vi "Resubscribe to Cloneable.vi"(8 "error in":errorcluster, 11 "Module ID":i32=-1) -> (0 "error out":errorcluster)   [LabVIEW 2026, in "Core.lvlib"]
doc: "_____\nCreated using DQMH Framework: Event Scripter 7.1.2.1547."
uses:
  Core.lvlib
  Resubscribe to Cloneable Argument--cluster.ctl
  replay/Replay/src/Libraries/Replay/Broadcast Events--cluster.ctl
  replay/Replay/src/Libraries/Replay/Did Init Argument--cluster.ctl
  replay/Replay/src/Libraries/Replay/Status Updated Argument--cluster.ctl
  replay/Replay/src/Libraries/Replay/Error Reported Argument--cluster.ctl
  replay/Replay/src/Libraries/Replay/Stop Argument--cluster.ctl
  replay/Replay/src/Libraries/Replay/Get Module Execution Status Argument--cluster.ctl
  replay/Replay/src/Libraries/Replay/Replay Finished Processing User Events Argument--cluster.ctl
  replay/Replay/src/Libraries/Replay/Load UserEvents (Reply Payload)--cluster.ctl
  replay/Replay/src/Libraries/User Events Metadata.ctl
  replay/Replay/src/Libraries/Replay/Replay.lvlib
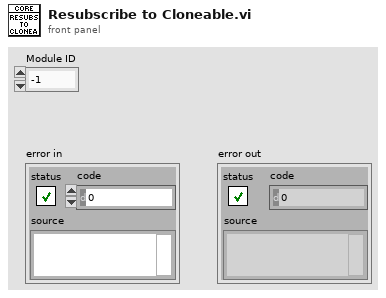
[diagram p1: front panel]
types:
  T1 = typedef "Replay.lvlib/Broadcast Events--cluster.ctl" = cluster{"Module Did Init":refnum<user-event>, "Status Updated":refnum<user-event>, "Error Reported":refnum<user-event>, "Module Did Stop":refnum<user-event>, "Update Module Execution Status":refnum<user-event>, "Replay Finished Processing User Events":refnum<user-event>, "User Events Metadata":refnum<user-event>}
  T2 = typedef "Core.lvlib/Resubscribe to Cloneable Argument--cluster.ctl" = cluster{"Module ID":i32, "Replay Broadcast Events":T1}
  T3 = typedef "Core.lvlib/Request Events--cluster.ctl" = cluster{"Stop Module":refnum<user-event>, "Show Panel":refnum<user-event>, "Hide Panel":refnum<user-event>, "Show Diagram":refnum<user-event>, "Get Module Execution Status":refnum<user-event>, "Resubscribe to Cloneable":refnum<user-event>, "LaunchReplayModule":refnum<user-event>, "Local Instance":T4, "Record Run ID":refnum<user-event>}
  T4 = typedef "Core.lvlib/Local Instance Request Events--cluster.ctl" = cluster{"Set Record Run ID":refnum<user-event>}
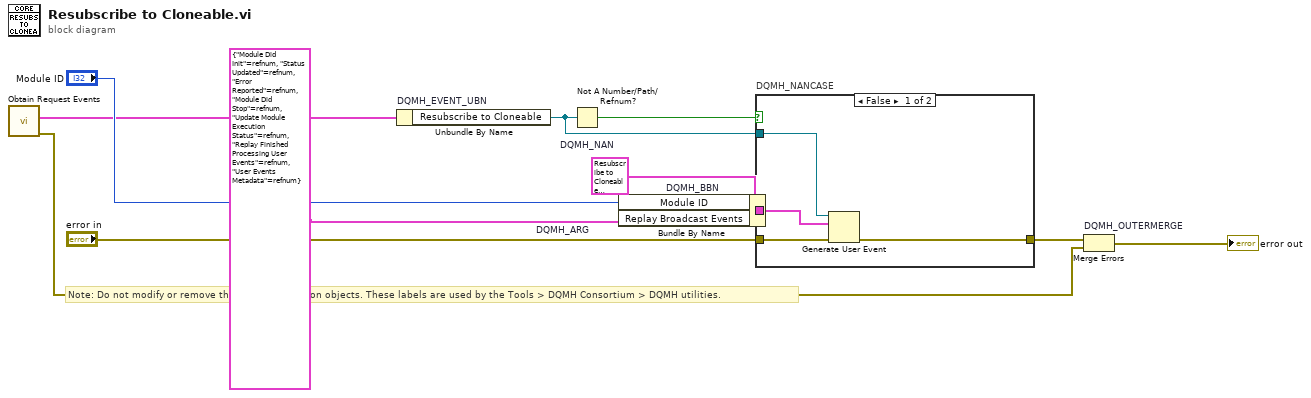
[diagram p0: block diagram]
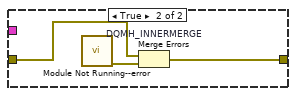
[diagram p2: hidden frame]
diagram:
  w5 = T2 {"Module ID"=-1, "Replay Broadcast Events"={"Module Did Init"=refnum, "Status Updated"=refnum, "Error Reported"=refnum, "Module Did Stop"=refnum, "Update Module Execution Status"=refnum, "Replay Finished Processing User Events"=refnum, "User Events Metadata"=refnum}}  # DQMH_ARG
  # "Note: Do not modify or remove the \"DQMH\" labels on objects. These labels are used by the Tools > DQMH Consortium > DQMH utilities."
  n1 = call "Obtain Request Events.vi"() -> ("error out"=w3:errorcluster, "Core Request Events"=w2:T3)  [unwired: 10 in]
  n2 = Unbundle By Name "DQMH_EVENT_UBN"(w2) -> ("Resubscribe to Cloneable"=w7:refnum<user-event>)
  n3 = Not A Number/Path/Refnum? "DQMH_NAN"(number/path/refnum=w7) -> (NaN/Path/Refnum?=w8:bool)
  n4 = Bundle By Name "DQMH_BBN"(cluster=w5, "Module ID"="Module ID", "Replay Broadcast Events"=T1 {"Module Did Init"=refnum, "Status Updated"=refnum, "Error Reported"=refnum, "Module Did Stop"=refnum, "Update Module Execution Status"=refnum, "Replay Finished Processing User Events"=refnum, "User Events Metadata"=refnum}) -> (w9:T2)
  n5 = case "DQMH_NANCASE" shown="False" w8 {
    tunnel: "error in" -> [w15 w18]
    tunnel: [w14 w17] -> w6
    tunnel: w7 -> [w13 _]
    tunnel: w9 -> [w12 _]
    frame False {
      n6 = Generate User Event(user event=w13, event data cluster=w12, error in=w15) -> (error out=w14:errorcluster)  [unwired: 1 in, 1 out]
    }
    frame True {
      n7 = call "Module Not Running--error.vi"() -> ("error out"=w16:errorcluster)  [unwired: 11 in]
      n8 = Merge Errors "DQMH_INNERMERGE"(w18, w16) -> (w17:errorcluster)
    }
  }
  n9 = Merge Errors "DQMH_OUTERMERGE"(w6, w3) -> (→"error out":errorcluster)
